vi "Kinect Global.vi"() -> ()   [LabVIEW 2014]
uses:
  Resources/Others/Control cluster.ctl
panel:
  in  "Calibrate Pitch":bool
  out "3D Picture":refnum<vi>(3d-picture)
  in  "pitch offset":dbl=0.15 format="%#_13g"
  out "Control Cluster":T1 {"Yaw Speed" scale=-1.0..1.0; "Vertical Speed" scale=-1.0..1.0; "Pitch" scale=-1.0..1.0; "Roll" scale=-1.0..1.0}
  in  "Weak detection/Error":bool=TRUE
  in  "Hover":bool=TRUE
  in  "Toggle Land/Take off":bool
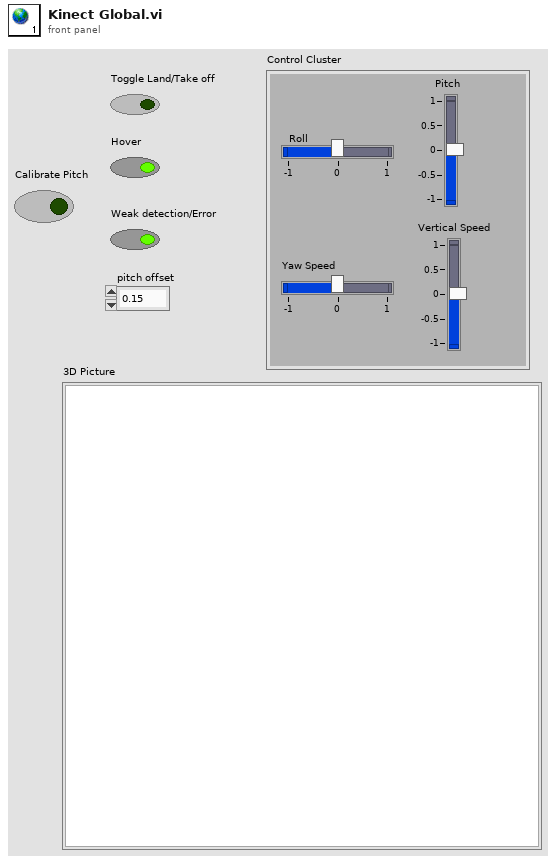
[diagram p1: front panel]
types:
  T1 = typedef "Control cluster.ctl" = cluster{"Roll":sgl, "Pitch":sgl, "Vertical Speed":sgl, "Yaw Speed":sgl}
diagram:
